vi "Init Control.vi"(5 "Group":refnum<class "Group DBL.lvclass">, 6 "Period ms":i64, 7 "VolatusAPI":refnum<class "VolatusAPI.lvclass">, 8 "error in (no error)":errorcluster, 9 "Control MsgQ":refnum<class "MessageQ.lvclass">, 10 "Config Element":refnum<class "Config Element.lvclass">, 11 "Valve in":refnum<class "BangBangControl.lvclass">) -> (0 "error out":errorcluster, 3 "Valve out":refnum<class "BangBangControl.lvclass">)   [LabVIEW 2020, in "VolatusControl.lvlib" / "BangBangControl.lvclass"]
uses:
  BangBangControl.lvclass
  lv-cdm/CDM-Config/Config Element/Config Element.lvclass
  Volatus/VolatusAPI/VolatusAPI.lvclass
  Volatus/MessageQ/MessageQ.lvclass
  lv-vecto/Vecto/Group DBL/Group DBL.lvclass
  C:/dev/lv20CE/relink/lv-vecto/Vecto/Group/Group.lvclass
  BangBangControl.lvclass/BangBangControl.ctl
  lv-cdm/CDM-Config/Config Element/Owner.vi
  lv-cdm/CDM-Config/Config Manager/Lookup Descendant.vi
  VolatusControl.lvlib
  lv-vecto/Vecto/Group/Group.lvclass
  lv-cdm/CDM-Config/Config Filter/Config Lookup.lvclass
  C:/dev/lv20CE/relink/lv-vecto/Vecto/Group DBL/Group DBL.lvclass
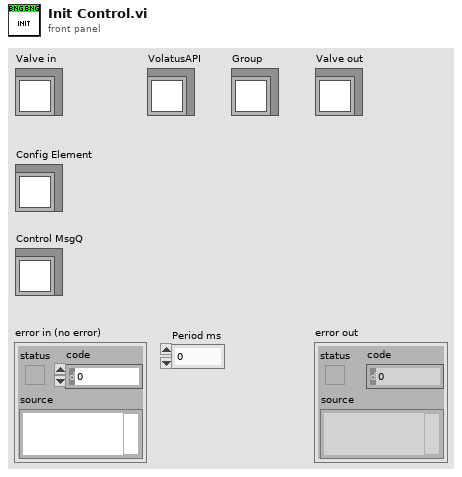
[diagram p1: front panel]
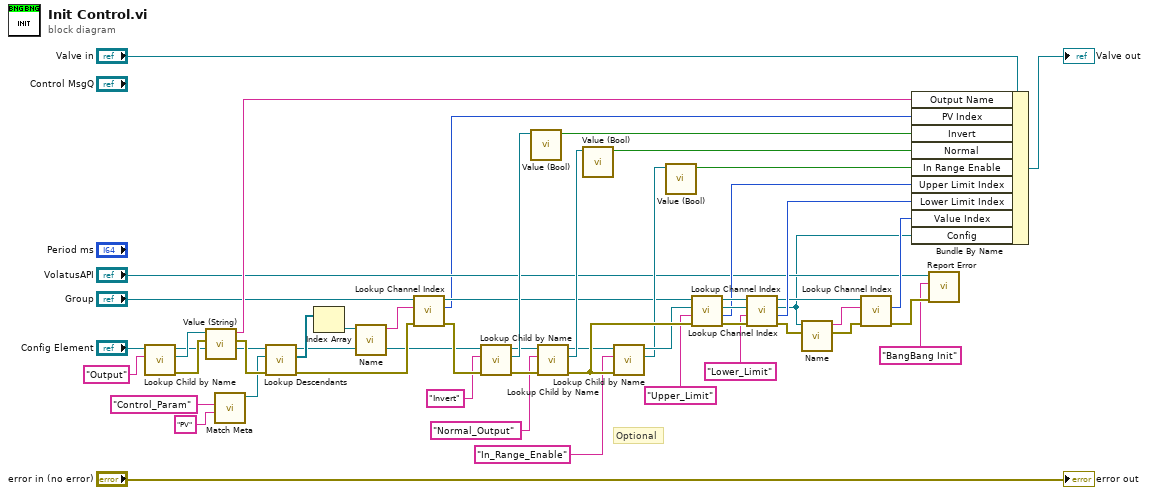
[diagram p0: block diagram]
diagram:
  # "Optional"
  n1 = call "Lookup Child by Name.vi"("Name"="Output", "Config Element in"="Config Element") -> ("error out"=w42:errorcluster, "Child"=w43:refnum<class "Config Element.lvclass">, "Config Element out"=w1:refnum<class "Config Element.lvclass">)  [unwired: 6 in, 1 out]
  n2 = call "Value (String).vi"("error in (no error)"=w42, "Config Element in"=w43) -> ("error out"=w52:errorcluster, "String Value"=w40:string)  [unwired: 8 in]
  n3 = call "Match Meta.vi"("Value (Any)"="PV" ("Name"), "Name"="Control_Param") -> ("Config Lookup out"=w10:refnum<class "Config Lookup.lvclass">)  [unwired: 8 in, 1 out]
  n4 = call "Lookup Descendants.vi"("error in (no error)"=w52, "Lookup"=w10, "Config Element in"=w1) -> ("error out"=w50:errorcluster, "Descendants"=w4:refnum<class "Config Element.lvclass">[], "Config Element out"=w3:refnum<class "Config Element.lvclass">)  [unwired: 6 in]
  n5 = Index Array(array=w4) -> (element=w9:refnum<class "Config Element.lvclass">)  [unwired: 1 in]
  n6 = call "Name.vi"("Config Element in"=w9) -> ("Name"=w8:string)  [unwired: 9 in, 1 out]
  n7 = call "Lookup Channel Index.vi"("error in (no error)"=w50, "Channel Name"=w8, "Group in"="Group") -> ("error out"=w51:errorcluster, "Index"=w5:i32, "Group out"=w6:refnum<class "Group DBL.lvclass">)  [unwired: 6 in]
  n8 = call "Lookup Child by Name.vi"("error in (no error)"=w51, "Name"="Invert", "Config Element in"=w3) -> ("error out"=w48:errorcluster, "Child"=w38:refnum<class "Config Element.lvclass">, "Config Element out"=w34:refnum<class "Config Element.lvclass">)  [unwired: 5 in, 1 out]
  n9 = call "Value (Bool).vi"("Config Element in"=w38) -> ("Bool Value"=w37:bool)  [unwired: 9 in, 1 out]
  n10 = call "Lookup Child by Name.vi"("error in (no error)"=w48, "Name"="Normal_Output", "Config Element in"=w34) -> ("error out"=w49:errorcluster, "Child"=w36:refnum<class "Config Element.lvclass">, "Config Element out"=w18:refnum<class "Config Element.lvclass">)  [unwired: 5 in, 1 out]
  n11 = call "Value (Bool).vi"("Config Element in"=w36) -> ("Bool Value"=w33:bool)  [unwired: 9 in, 1 out]
  n12 = call "Lookup Child by Name.vi"("error in (no error)"=w49, "Name"="In_Range_Enable", "Config Element in"=w18) -> ("Child"=w15:refnum<class "Config Element.lvclass">, "Config Element out"=w16:refnum<class "Config Element.lvclass">)  [unwired: 5 in, 2 out]
  n13 = call "Value (Bool).vi"("Config Element in"=w15) -> ("Bool Value"=w14:bool)  [unwired: 9 in, 1 out]
  n14 = call "Lookup Channel Index.vi"("error in (no error)"=w49, "Meta Value"="Upper_Limit", "Config Element in"=w16, "Group in"=w6) -> ("error out"=w30:errorcluster, "Index"=w28:i32, "Config Element"=w29:refnum<class "Config Element.lvclass">, "Group"=w31:refnum<class "Group DBL.lvclass">)  [unwired: 4 in]
  n15 = call "Lookup Channel Index.vi"("error in (no error)"=w30, "Meta Value"="Lower_Limit", "Config Element in"=w29, "Group in"=w31) -> ("error out"=w22:errorcluster, "Index"=w26:i32, "Config Element"=w2:refnum<class "Config Element.lvclass">, "Group"=w23:refnum<class "Group DBL.lvclass">)  [unwired: 4 in]
  n16 = call "Name.vi"("error in (no error)"=w22, "Config Element in"=w2) -> ("error out"=w24:errorcluster, "Name"=w25:string)  [unwired: 8 in]
  n17 = call "Lookup Channel Index.vi"("error in (no error)"=w24, "Channel Name"=w25, "Group in"=w23) -> ("error out"=w20:errorcluster, "Index"=w21:i32)  [unwired: 6 in, 1 out]
  n18 = Bundle By Name(cluster="Valve in", "Output Name"=w40, "PV Index"=w5, "Invert"=w37, "Normal"=w33, "In Range Enable"=w14, "Upper Limit Index"=w28, "Lower Limit Index"=w26, "Value Index"=w21, "Config"=w2) -> (→"Valve out":refnum<class "BangBangControl.lvclass">)
  n19 = call "Report Error.vi"("error in (no error)"=w20, "Context"="BangBang Init", "VolatusAPI in"="VolatusAPI") -> ()  [unwired: 7 in, 2 out]
  "error out" <- "error in (no error)"
